vi "FP Layout Dual.vi"() -> ()   [LabVIEW 2026]
doc: "Scripting helper (not part of the application). Opens a VI by path and walks its front-panel controls. Read pass (Apply false): returns each control's label, position and size. Apply pass: moves each control named in Names to (Left, Top), sizes the plot area of each graph named in Graph Names, sets its Y-scale name, sets the panel window bounds and saves the VI."
panel:
  out "error out":errorcluster
  out "Heights":i32[](array[numeric])
  out "Widths":i32[](array[numeric])
  out "Tops":i32[](array[numeric])
  out "Lefts":i32[](array[numeric])
  out "Labels":string[](array[string])
  in  "error in":errorcluster
  in  "Apply":bool
  in  "vi path":string
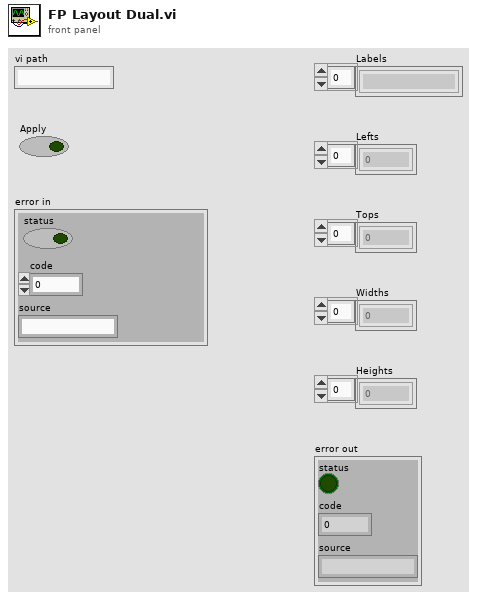
[diagram p1: front panel]
types:
  T1 = cluster{"Left":i32, "Top":i32, "Right":i32, "Bottom":i32}
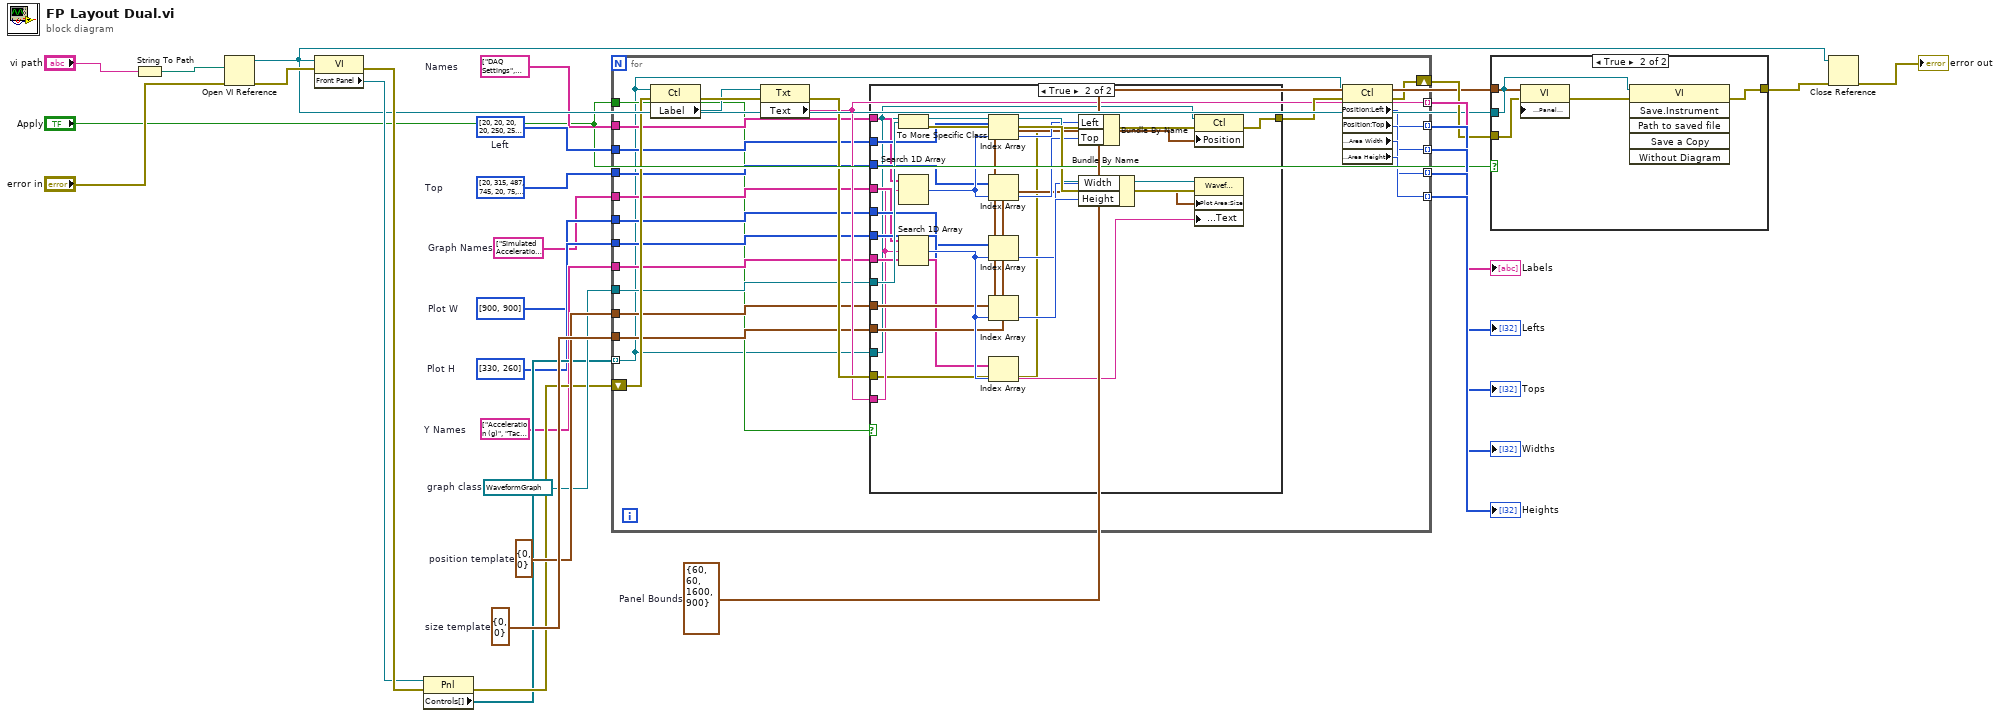
[diagram p0: block diagram]
diagram:
  w21 = cluster{"Width":i32, "Height":i32} {"Width"=0, "Height"=0}  # size template
  w20 = cluster{"Left":i32, "Top":i32} {"Left"=0, "Top"=0}  # position template
  w19 = refnum<vi> refnum  # graph class
  w10 = T1 {"Left"=60, "Top"=60, "Right"=1600, "Bottom"=900}  # Panel Bounds
  w9 = string[] ["Acceleration (g)", "Tach (V)"]  # Y Names
  w8 = i32[] [330, 260]  # Plot H
  w7 = i32[] [900, 900]  # Plot W
  w6 = string[] ["Simulated Acceleration (g)", "Tach Output (V)"]  # Graph Names
  w5 = i32[] [20, 315, 487, 745, 20, 75, 490, 20, 500, 20]  # Top
  w4 = i32[] [20, 20, 20, 20, 250, 250, 250, 1230, 1230, 1375]  # Left
  w3 = string[] ["DAQ Settings", "Tach Output", "Speed Profile", "STOP", "Shaft Speed (rpm)", "Simulated Acceleration (g)", "Tach Output (V)", "Fault Injection", "Fault Frequencies (Hz)", "Sim Config"]  # Names
  n1 = String To Path(string="vi path") -> (path=w12:path)
  n2 = Open VI Reference(vi path=w12, error in (no error)="error in") -> (vi reference=w13:refnum<vi>, error out=w14:errorcluster)  [unwired: 4 in]
  n3 = property class="VI"(reference=w13, error in=w14) -> (error out=w16:errorcluster, "Front Panel"=w15:refnum<vi>)  [unwired: 1 out]
  n4 = property class="Pnl"(reference=w15, error in=w16) -> (error out=w18:errorcluster, "Controls[]"=w17:refnum<vi>[])  [unwired: 1 out]
  n5 = for {
    tunnel: "Apply" -> [w31]
    tunnel: w3 -> [w32]
    tunnel: w4 -> [w33]
    tunnel: w5 -> [w34]
    tunnel: w6 -> [w35]
    tunnel: w7 -> [w36]
    tunnel: w8 -> [w37]
    tunnel: w9 -> [w38]
    tunnel: w19 -> [w39]
    tunnel: w20 -> [w40]
    tunnel: w21 -> [w41]
    tunnel: w17 -> [w30] mode=indexing
    shift-right: [w43] -> w22
    shift-left: w18 -> [w42]
    tunnel: [w46] -> w23 mode=indexing
    tunnel: [w49] -> w24 mode=indexing
    tunnel: [w50] -> w25 mode=indexing
    tunnel: [w51] -> w26 mode=indexing
    tunnel: [w52] -> w27 mode=indexing
    n6 = property class="Ctl"(reference=w30, error in=w42) -> (error out=w45:errorcluster, "Label"=w44:refnum<vi>)  [unwired: 1 out]
    n7 = property class="Txt"(reference=w44, error in=w45) -> (error out=w47:errorcluster, "Text"=w46:string)  [unwired: 1 out]
    n8 = case shown="True" w31 {
      tunnel: w32 -> [_ w57]
      tunnel: w33 -> [_ w58]
      tunnel: w34 -> [_ w59]
      tunnel: w35 -> [_ w60]
      tunnel: w36 -> [_ w61]
      tunnel: w37 -> [_ w62]
      tunnel: w38 -> [_ w63]
      tunnel: w39 -> [_ w64]
      tunnel: w40 -> [_ w65]
      tunnel: w41 -> [_ w66]
      tunnel: w30 -> [_ w54]
      tunnel: w47 -> [w53 w55]
      tunnel: w46 -> [_ w56]
      tunnel: [w53 w71] -> w48
      frame False {
      }
      frame True {
        n9 = To More Specific Class(target class=w64, reference=w54) -> (specific class reference=w77:refnum<vi>, error out=w78:errorcluster)  [unwired: 1 in]
        n10 = Search 1D Array(1D array=w57, element=w56) -> (index of element=w67:i32)  [unwired: 1 in]
        n11 = Search 1D Array(1D array=w60, element=w56) -> (index of element=w72:i32)  [unwired: 1 in]
        n12 = Index Array(array=w58, index=w67) -> (element=w68:i32)
        n13 = Index Array(array=w59, index=w67) -> (element=w69:i32)
        n14 = Index Array(array=w61, index=w72) -> (element=w73:i32)
        n15 = Index Array(array=w62, index=w72) -> (element=w74:i32)
        n16 = Index Array(array=w63, index=w72) -> (element=w75:string)
        n17 = Bundle By Name(cluster=w65, "Left"=w68, "Top"=w69) -> (w70:cluster{"Left":i32, "Top":i32})
        n18 = Bundle By Name(cluster=w66, "Width"=w73, "Height"=w74) -> (w76:cluster{"Width":i32, "Height":i32})
        n19 = property class="Ctl"(reference=w54, error in=w55, "Position"=w70) -> (error out=w71:errorcluster)  [unwired: 1 out]
        n20 = property class="WaveformGraph (strict)"(reference=w77, error in=w78, "Plot Area:Size"=w76, "Y Scale.Name Label.Text"=w75) -> ()  [unwired: 2 out]
      }
    }
    n21 = property class="Ctl"(reference=w30, error in=w48) -> (error out=w43:errorcluster, "Position:Left"=w49:i32, "Position:Top"=w50:i32, "Bounds:Area Width"=w51:u32, "Bounds:Area Height"=w52:u32)  [unwired: 1 out]
  }
  "Labels" <- w23
  "Lefts" <- w24
  "Tops" <- w25
  "Widths" <- w26
  "Heights" <- w27
  n22 = case shown="True" "Apply" {
    tunnel: w10 -> [_ w82]
    tunnel: w13 -> [_ w80]
    tunnel: w22 -> [w79 w81]
    tunnel: [w79 w84] -> w28
    frame False {
    }
    frame True {
      n23 = property class="VI"(reference=w80, error in=w81, "Front Panel Window:Panel Bounds"=w82) -> (error out=w83:errorcluster)  [unwired: 1 out]
      n24 = invoke class="VI" method="Save.Instrument"(reference=w80, error in=w83) -> (error out=w84:errorcluster)  [unwired: 4 in, 5 out]
    }
  }
  n25 = Close Reference(reference=w13, error in (no error)=w28) -> (error out=→"error out":errorcluster)
